vi "Insert into Subpanel.vi"(8 "error in (no error)":errorcluster, 10 "SubPanel":refnum<vi>, 11 "Missing VI Type in":refnum<class "Missing VI Type.lvclass">) -> (0 "error out":errorcluster, 3 "Missing VI Type out":refnum<class "Missing VI Type.lvclass">)   [LabVIEW 2020, in "Peek Window.lvlib" / "Missing VI Type.lvclass"]
uses:
  Missing VI Type.lvclass
  D:/Code/VI-Peek/source/Peek Window/VI Types/Standard VI Type/Standard VI Type.lvclass
  Standard VI Type/Standard VI Type.lvclass/Standard VI Type.ctl
  Missing VI Type.lvclass/Missing VI Type.ctl
  Standard VI Type/Read Full Qualified Name.vi
  Missing VI Message.vi
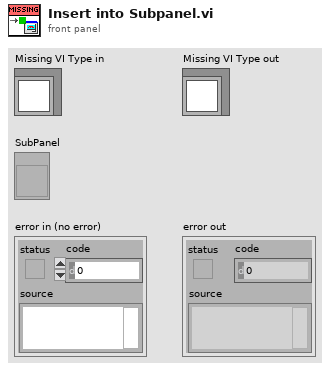
[diagram p1: front panel]
types:
  T1 = enum8{"Enabled", "Disabled", "Disabled and Grayed Out"}
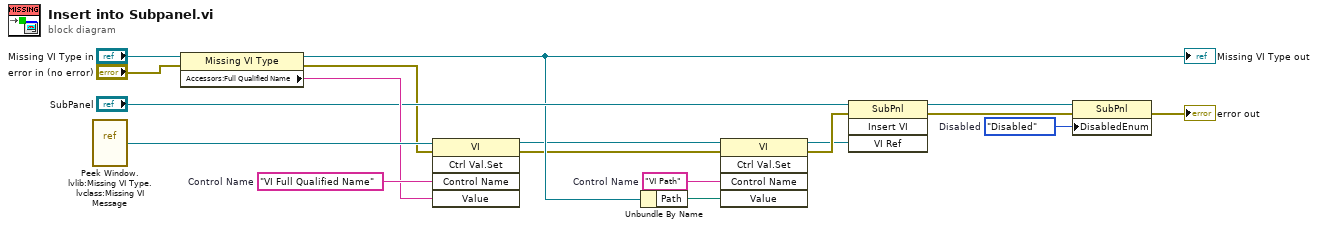
[diagram p0: block diagram]
diagram:
  w3 = T1."Disabled"  # Disabled
  w13 = "VI Path"  # Control Name
  w17 = "VI Full Qualified Name"  # Control Name
  n1 = vi-ref "Peek Window.lvlib:Missing VI Type.lvclass:Missing VI Message.vi"() -> (w16:refnum<vi>)
  n2 = property class="Missing VI Type"(reference="Missing VI Type in", error in="error in (no error)") -> (reference out=w12:refnum<class "Missing VI Type.lvclass">, error out=w1:errorcluster, "Accessors:Full Qualified Name"=w15:string)
  "Missing VI Type out" <- w12
  n3 = invoke class="VI" method="Ctrl Val.Set"(reference=w16, error in=w1, "Control Name"=w17, "Value"=w15) -> (reference out=w10:refnum<vi>, error out=w9:errorcluster)  [unwired: 1 in, 3 out]
  n4 = Unbundle By Name(w12) -> ("Path"=w11:path)
  n5 = invoke class="VI" method="Ctrl Val.Set"(reference=w10, error in=w9, "Control Name"=w13, "Value"=w11) -> (reference out=w7:refnum<vi>, error out=w8:errorcluster)  [unwired: 1 in, 3 out]
  n6 = invoke class="SubPnl" method="Insert VI"(reference="SubPanel", error in=w8, "VI Ref"=w7) -> (reference out=w5:refnum<vi>, error out=w6:errorcluster)  [unwired: 1 in, 2 out]
  n7 = property class="SubPnl"(reference=w5, error in=w6, "DisabledEnum"=w3) -> (error out=→"error out":errorcluster)  [unwired: 1 out]
